vi "removeChild.vi"(0 "reference":refnum<class "AbstractNode.lvclass">, 1 "node":refnum<class "AbstractNode.lvclass">, 5 "error in (no error)":errorcluster) -> (14 "reference out":refnum<class "AbstractNode.lvclass">, 19 "error out":errorcluster)   [LabVIEW 2020, in "AbstractNode.lvclass"]
doc: "public void removeChild(Node node)"
uses:
  <resource>/Framework/Providers/Open_GDS/UML/AbstractNode_class/AbstractNode.lvclass
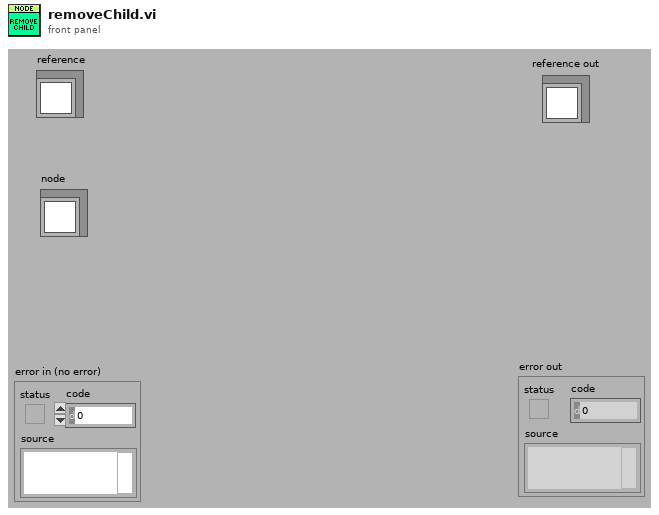
[diagram p1: front panel]
types:
  T1 = typedef "AbstractNode.lvclass/ObjectAttributes.ctl" = cluster{"parent":refnum<class "AbstractNode.lvclass">, "children":refnum<class "AbstractNode.lvclass">[], "Hidden":bool}
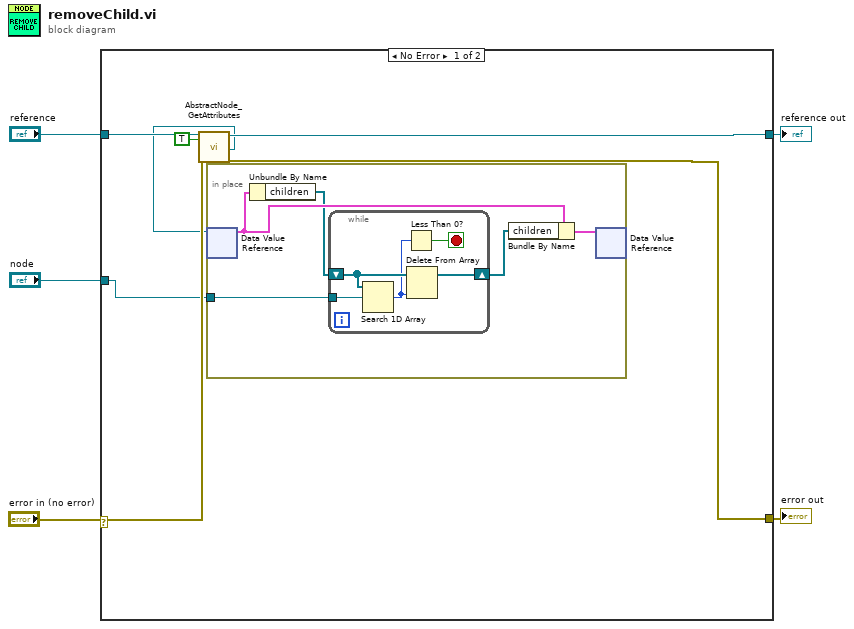
[diagram p0: block diagram]
diagram:
  n1 = case shown="No Error" "error in (no error)" {
    selector: "error in (no error)" -> [w9 w23]
    tunnel: "reference" -> [w12 w24]
    tunnel: [w11 w23] -> w4
    tunnel: [w10 w24] -> w3
    tunnel: "node" -> [w6 _]
    frame No Error {
      n2 = call <resource>:"AbstractNode_GetAttributes.vi"("reference in"=w12, "OnlyGetDvrReference(False)"=TRUE, "error in (no error)"=w9) -> ("reference out"=w10:refnum<class "AbstractNode.lvclass">, "DataRef"=w7:refnum<data-value>, "error out"=w11:errorcluster)  [unwired: 13 in, 1 out]
      n3 = in-place {
        in-place-border: w6 -> [w13]
        n4 = in-place-dvr #1(w7) -> (w17:T1)  [unwired: 1 out]
        n5 = Unbundle By Name(w17) -> ("children"=w14:refnum<class "AbstractNode.lvclass">[])
        n6 = while {
          tunnel: w13 -> [w22]
          shift-right: [w21] -> w16
          shift-left: w14 -> [w20]
          stop <- w18 stop-if-true
          n7 = Search 1D Array(1D array=w20, element=w22) -> (index of element=w19:i32)  [unwired: 1 out]
          n8 = Less Than 0?(x=w19) -> (x < 0?=w18:bool)
          n9 = Delete From Array(array=w20, index=w19) -> (array with subset deleted=w21:refnum<class "AbstractNode.lvclass">[])  [unwired: 1 in, 1 out]
        }
        n10 = Bundle By Name(cluster=w17, "children"=w16) -> (w15:T1)
        n11 = in-place-dvr #1(w15) -> ()  [unwired: 2 out]
      }
    }
    frame Error {
    }
  }
  "reference out" <- w3
  "error out" <- w4
